vi "Module Init.vi"(8 "error in (no error)":errorcluster, 11 "Data Logger Module in":refnum<class "Data Logger DBL Module.lvclass">) -> (0 "error out":errorcluster, 3 "Data Logger Module out":refnum<class "Data Logger DBL Module.lvclass">)   [LabVIEW 2020, in "VolatusData.lvlib" / "Data Logger DBL Module.lvclass"]
uses:
  Data Logger DBL Module.lvclass
  C:/dev/lv20CE/relink/lv-volatus/Volatus/Module/Module.lvclass
  Volatus/Module/Module.lvclass/Module.ctl
  Register Logger.ctl
  Volatus/MessageQ/MessageQ.lvclass
  Logger State.ctl
  Data Logger DBL Module.lvclass/Data Logger DBL Module.ctl
  Volatus/MessageQ/MessageQ.lvclass/MessageQ.ctl
  Log Manager Identity/Log Manager Identity.lvclass
  C:/dev/lv20CE/relink/lv-volatus/Volatus/Identity/Identity.lvclass
  Volatus/Module/Update Substatus.vi
  Volatus/VolatusAPI/VolatusAPI.lvclass
  Volatus/Module/Module.lvclass
  VolatusData.lvlib
  C:/dev/lv20CE/relink/lv-volatus/VolatusData/Data Logger DBL Module/Data Logger DBL Module.lvclass
  C:/dev/lv20CE/relink/lv-volatus/VolatusData/Log Manager Identity/Log Manager Identity.lvclass
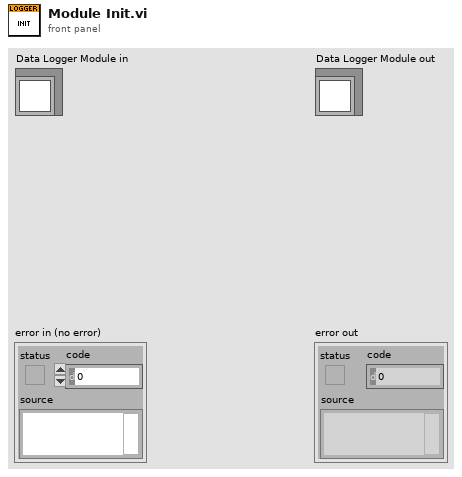
[diagram p1: front panel]
types:
  T1 = typedef "VolatusData.lvlib/Register Logger.ctl" = cluster{"MsgQ":refnum<class "MessageQ.lvclass">, "ID":string, "Group":string}
  T2 = typedef "VolatusData.lvlib/Logger State.ctl" = enum16{"Unknown", "Idle", "Preparing", "Ready", "Logging", "Stopping"}
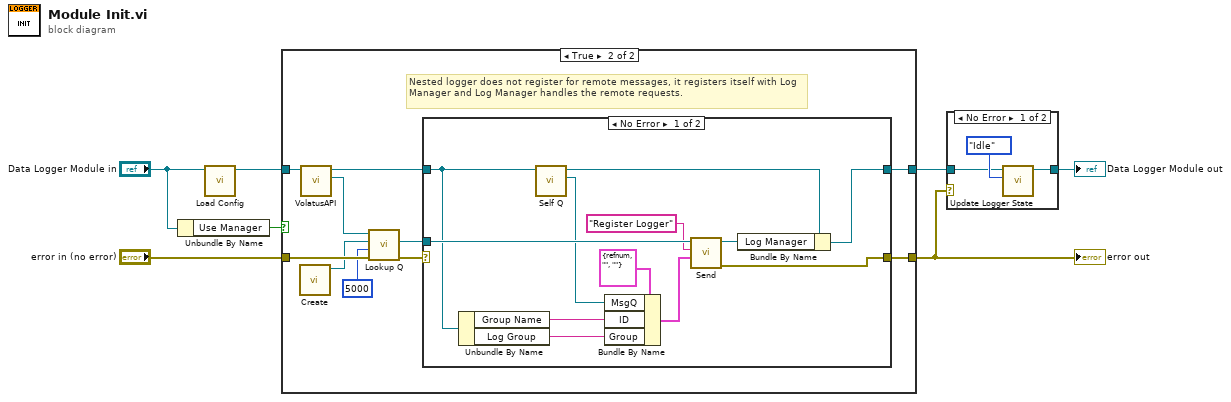
[diagram p0: block diagram]
diagram:
  n1 = Unbundle By Name("Data Logger Module in") -> ("Use Manager"=w3:bool)
  n2 = call "Load Config.vi"("Data Logger Module in"="Data Logger Module in") -> ("Data Logger Module out"=w1:refnum<class "Data Logger DBL Module.lvclass">)  [unwired: 9 in, 1 out]
  n3 = case shown="True" w3 {
    tunnel: "error in (no error)" -> [w8 w19]
    tunnel: w1 -> [w9 w17]
    tunnel: [w9 w12] -> w6
    tunnel: [w8 w11] -> w4
    frame False {
      # "False was passed in for Use Manager input in Create.vi so that the logger can be used more directly."
    }
    frame True {
      # "Nested logger does not register for remote messages, it registers itself with Log Manager and Log Manager handles the remote requests."
      n4 = call "Create.vi"() -> ("Log Manager Identity out"=w15:refnum<class "Log Manager Identity.lvclass">)  [unwired: 11 in]
      n5 = call "VolatusAPI.vi"("Module in"=w17) -> ("VolatusAPI"=w16:refnum<class "VolatusAPI.lvclass">, "Module out"=w10:refnum<class "Data Logger DBL Module.lvclass">)  [unwired: 9 in]
      n6 = call "Lookup Q.vi"("error in (no error)"=w19, "Timeout ms (0)"=5000, "Identity"=w15, "VolatusAPI in"=w16) -> ("error out"=w14:errorcluster, "MessageQ"=w13:refnum<class "MessageQ.lvclass">)  [unwired: 5 in, 1 out]
      n7 = case shown="No Error" w14 {
        selector: w14 -> [_ w33]
        tunnel: w13 -> [w31 _]
        tunnel: w10 -> [w23 w32]
        tunnel: [w21 w32] -> w12
        tunnel: [w25 w33] -> w11
        frame No Error {
          n8 = Unbundle By Name(w23) -> ("Group Name"=w20:string, "Log Group"=w22:string)
          n9 = call "Self Q.vi"("Module in"=w23) -> ("Self Q"=w27:refnum<class "MessageQ.lvclass">, "Module out"=w26:refnum<class "Data Logger DBL Module.lvclass">)  [unwired: 9 in]
          n10 = Bundle By Name(cluster=T1 {"MsgQ"=refnum, "ID"="", "Group"=""} ("Logger Registration"), "MsgQ"=w27, "ID"=w20, "Group"=w22) -> (w28:T1)
          n11 = call "Send.vi"("Data"=w28, "ID"="Register Logger", "MessageQ in"=w31) -> ("error out"=w25:errorcluster, "MessageQ out"=w24:refnum<class "MessageQ.lvclass">)  [unwired: 7 in]
          n12 = Bundle By Name(cluster=w26, "Log Manager"=w24) -> (w21:refnum<class "Data Logger DBL Module.lvclass">)
        }
        frame Error {
        }
      }
    }
  }
  "error out" <- w4
  n13 = case shown="No Error" w4 {
    tunnel: w6 -> [w35 w37]
    tunnel: [w34 w37] -> w5
    frame No Error {
      n14 = call "Update Logger State.vi"("Logger State"=Logger_State."Idle", "Module in"=w35) -> ("Module"=w34:refnum<class "Data Logger DBL Module.lvclass">)  [unwired: 8 in, 1 out]
    }
    frame Error {
    }
  }
  "Data Logger Module out" <- w5
